vi "Device Name Extract.vi"(11 ".pinmap File Path":path) -> (3 "Device Name":string)   [LabVIEW 2025, in "Digital Pattern Sequencer.lvclass"]
uses:
  Digital Pattern Sequencer.lvclass
  Digital Pattern Sequencer.lvclass/Digital Pattern Sequencer.ctl
  <vilib>/xml/NI_XML.lvlib
  <vilib>/xml/Load XML String.vi
  <resource>/objmgr/DOMUserDefRef.rc
  <vilib>/xml/XPath/Get All Matched Nodes (String).vi
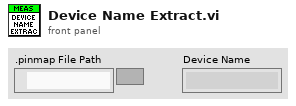
[diagram p1: front panel]
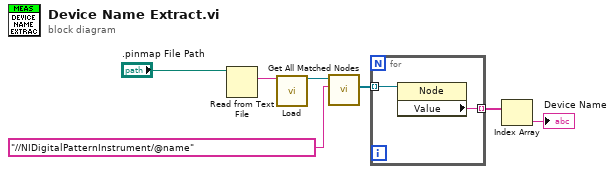
[diagram p0: block diagram]
diagram:
  n1 = Read from Text File(file (use dialog)=".pinmap File Path") -> (text=w6:string)  [unwired: 3 in, 3 out]
  n2 = call-poly <vilib>:"Load.vi"("XML string"=w6) -> ("DOM document out"=w7:refnum<k20>)  [unwired: 12 in, 2 out]
  n3 = call-poly <vilib>:"Get All Matched Nodes.vi"("XPath expression"="//NIDigitalPatternInstrument/@name", "node in"=w7) -> ("node result array"=w2:refnum<k20>[])  [unwired: 7 in, 2 out]
  n4 = for {
    tunnel: w2 -> [w9] mode=indexing
    tunnel: [w8] -> w3 mode=indexing
    n5 = property class="Node"(reference=w9) -> ("Value"=w8:string)  [unwired: 1 in, 2 out]
  }
  n6 = Index Array(array=w3) -> (element=→"Device Name":string)  [unwired: 1 in]
